vi "VM Spy - Truncate string value for list.vi"(10 "max length (40)":i32=40, 11 "String in":string) -> (3 "String out":string)   [LabVIEW 2021]
doc: "::: CalcExpress Toolkit :::\nCopyright (c) 2000-2026 Konstantin Shifershteyn. All rights reserved."
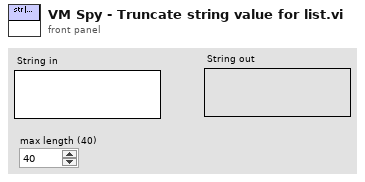
[diagram p1: front panel]
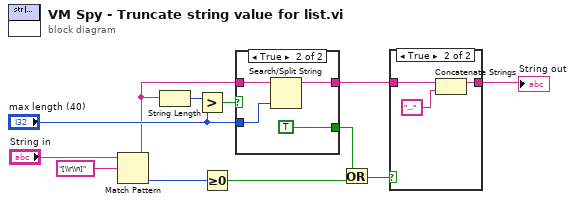
[diagram p0: block diagram]
diagram:
  n1 = Match Pattern(string="String in", regular expression="[\\r\\n]") -> (before substring=w5:string, offset past match=w10:i32)  [unwired: 1 in, 2 out]
  n2 = String Length(string=w5) -> (length=w7:i32)
  n3 = Greater?(x=w7, y="max length (40)") -> (0:w4:bool)
  n4 = Greater Or Equal To 0?(x=w10) -> (x >= 0?=w11:bool)
  n5 = case shown="True" w4 {
    tunnel: "max length (40)" -> [_ w17]
    tunnel: w5 -> [w13 w16]
    tunnel: [w13 w15] -> w2
    tunnel: [_ TRUE] -> w3
    frame False {
    }
    frame True {
      n6 = Search/Split String(string=w16, offset (0)=w17) -> (substring before match=w15:string)  [unwired: 1 in, 2 out]
    }
  }
  n7 = Or(x=w3, y=w11) -> (x .or. y?=w12:bool)
  n8 = case shown="True" w12 {
    tunnel: w2 -> [w18 w21]
    tunnel: [w18 w19] -> w1
    frame False {
    }
    frame True {
      n9 = Concatenate Strings(w21, "...") -> (w19:string)
    }
  }
  "String out" <- w1
